vi "classify error.vi"(8 "error to classify":errorcluster, 11 "SystemLin Tag Module runtime in":refnum<class "SystemLink runtime.lvclass">) -> (0 "classified error":errorcluster, 2 "error classification":T1, 3 "SystemLin Tag Module runtime out":refnum<class "SystemLink runtime.lvclass">)   [LabVIEW 2015, in "SystemLink runtime.lvclass"]
doc: "Allows a module to classify an error generated at any point during execution. This <b>error classification</b> can then be used by calling code to determine if execution can continue. In addition, this function can be used to allow a component to clear an error, convert an error to a warning, or attempt to recover from an error. Recovery may be attempted only if <b>attempt recovery?</b> is true."
uses:
  SystemLink runtime.lvclass
  <vilib>/NI/Tag Bus Module Framework/runtime/error classification.ctl
  <vilib>/NI/Tag Bus Module Framework/runtime/TBM module execution interface.lvclass
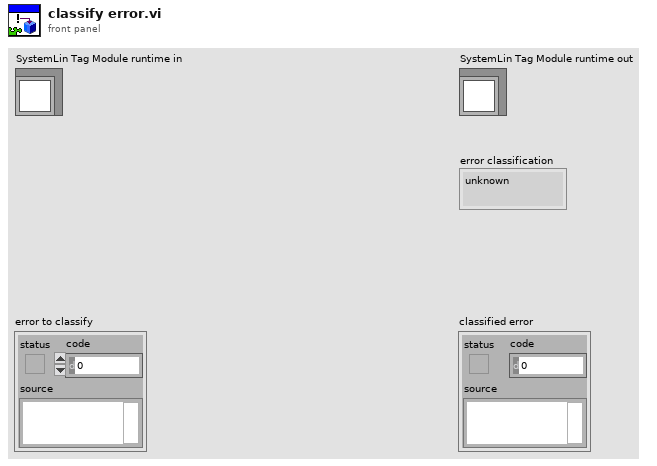
[diagram p1: front panel]
types:
  T1 = typedef "TBM module execution interface.lvclass/error classification.ctl" = enum16{"unknown", "none", "trivial", "recoverable", "critical"}
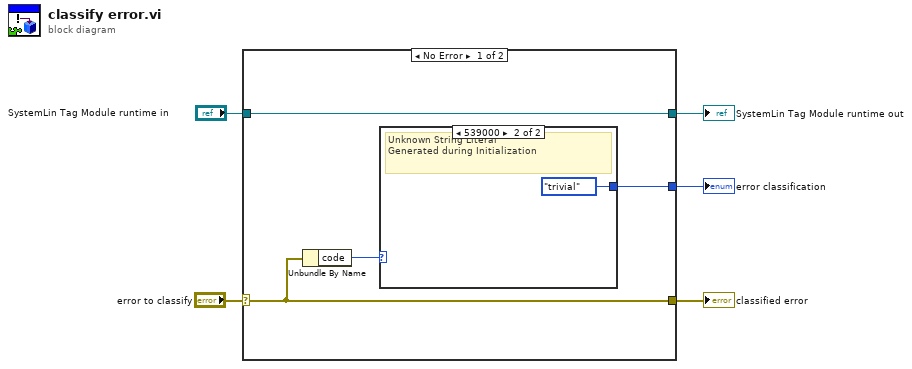
[diagram p0: block diagram]
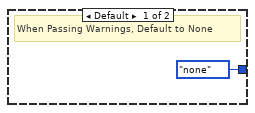
[diagram p2: hidden frame]
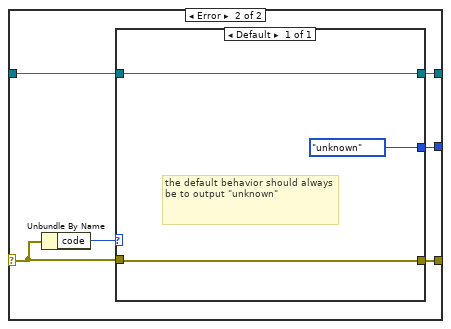
[diagram p3: hidden frame]
diagram:
  n1 = case shown="No Error" "error to classify" {
    selector: "error to classify" -> [w7 w16]
    tunnel: [w9 w12] -> w4
    tunnel: "SystemLin Tag Module runtime in" -> [w9 w13]
    tunnel: [w7 w15] -> w2
    tunnel: [w8 w14] -> w1
    frame No Error {
      n2 = Unbundle By Name(w7) -> ("code"=w6:i32)
      n3 = case shown="539000" w6 {
        tunnel: [error_classification."none" ("error classification") error_classification."trivial" ("error classification")] -> w8
        frame Default {
          # "When Passing Warnings, Default to None"
        }
        frame 539000 {
          # "Unknown String Literal\nGenerated during Initialization"
        }
      }
    }
    frame Error {
      n4 = Unbundle By Name(w16) -> ("code"=w17:i32)
      n5 = case shown="Default" w17 {
        tunnel: w16 -> [w18]
        tunnel: [w18] -> w15
        tunnel: [error_classification."unknown" ("error classification")] -> w14
        tunnel: w13 -> [w19]
        tunnel: [w19] -> w12
        frame Default {
          # "the default behavior should always be to output \"unknown\""
        }
      }
    }
  }
  "SystemLin Tag Module runtime out" <- w4
  "error classification" <- w1
  "classified error" <- w2
